vi "read_c_string_at_memory_address.vi"(6 "string_length":u64, 8 "error in (no error)":errorcluster, 11 "memory_address":u64) -> (0 "error out":errorcluster, 2 "data":u8[](array[numeric]), 3 "memory_address out":u64)   [LabVIEW 2020, in "reqwest.lvlib"]
uses:
  reqwest.lvlib
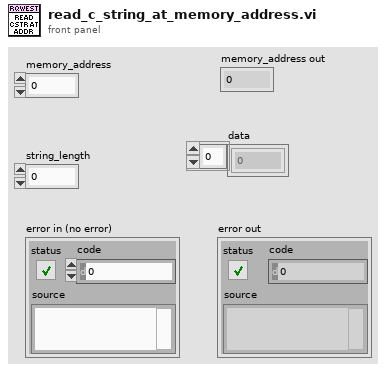
[diagram p1: front panel]
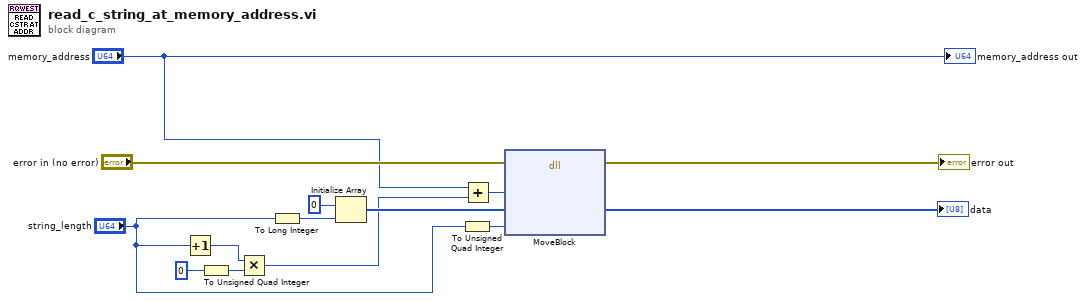
[diagram p0: block diagram]
diagram:
  n1 = Increment(x="string_length") -> (x+1=w11:u64)
  n2 = To Unsigned Quad Integer(1:u64 0 ("number")) -> (0:w5:u64)
  n3 = Multiply(x=w11, y=w5) -> (x*y=w6:u64)
  n4 = To Long Integer(number="string_length") -> (32bit integer=w7:i32)
  n5 = Initialize Array(u8 0, w7) -> (w8:u8[])
  n6 = To Unsigned Quad Integer(1:"string_length") -> (0:w3:u64)
  n7 = Add(x="memory_address", y=w6) -> (x+y=w10:u64)
  n8 = dll-call lib="LabVIEW" fn="MoveBlock"(error in="error in (no error)", "src"=w10, "dst"=w8, "size"=w3) -> (error out=→"error out":errorcluster, "dst"=→"data":u8[])  [unwired: 5 in, 1 out]
  "memory_address out" <- "memory_address"
